vi "ISP Exmpl - Controls Container.vi"() -> ()   [LabVIEW 2021]
doc: "::: CalcExpress Toolkit :::\nCopyright (c) 2000-2026 Konstantin Shifershteyn. All rights reserved."
panel:
  in  "PATH":path=path "C:/"
  in  "ENUM":T1(ring)=enum."selection 2"
  in  "RING":u16(ring)=1 items=["value 0", "value 1", "value 2", "value 3", "value 4", "value 5"]
  in  "BOOL":bool=TRUE
  in  "A1DBL":dbl[](array[numeric])=[1.0, 2.0, 3.0, 4.0, 5.0]
  in  "CDB":cdb=-10.0+5.5i
  in  "DBL":dbl=3.14
  in  "STR":string="Hello world"
  in  "stop":bool
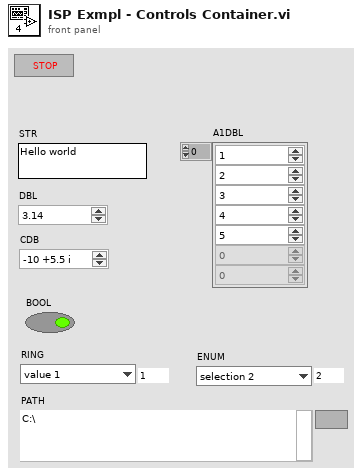
[diagram p1: front panel]
types:
  T1 = enum16{"selection 0", "selection 1", "selection 2", "selection 3", "selection 4", "selection 5", "selection 6"}
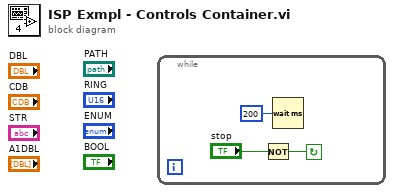
[diagram p0: block diagram]
diagram:
  n1 = while {
    stop <- w1 continue-if-true
    n2 = Not(x="stop") -> (.not. x?=w1:bool)
    n3 = Wait (ms)(milliseconds to wait=u32 200) -> ()  [unwired: 1 out]
  }
